vi "Build Toast With Classes.vi"(8 "error in":errorcluster) -> (0 "error out":errorcluster, 3 "Toast XML":string)   [LabVIEW 2026]
doc: "Interactive example using the public classes. Create a builder, add text, a Reply text input and a Reply button, inspect XML, initialize the service, register an injected ActivationHandler, then show the toast. Type a reply and click the toast button to inspect Arguments and User Inputs. Press Stop to unregister and close resources. A final System.GC.Collect call releases the callback reservation observed on this workstation; it is outside the callback. Running this VI displays a Windows notification and the example handler opens a blocking dialog."
uses:
  ActivationHandler/ActivationHandler.lvclass
  ToastBuilder/ToastBuilder.lvclass
  ToastService/ToastService.lvclass
panel:
  in  "stop":bool
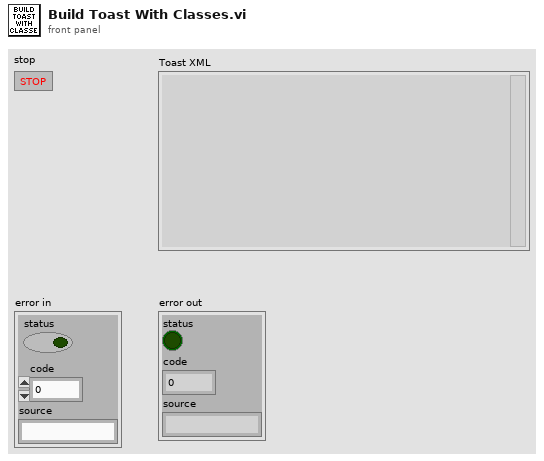
[diagram p1: front panel]
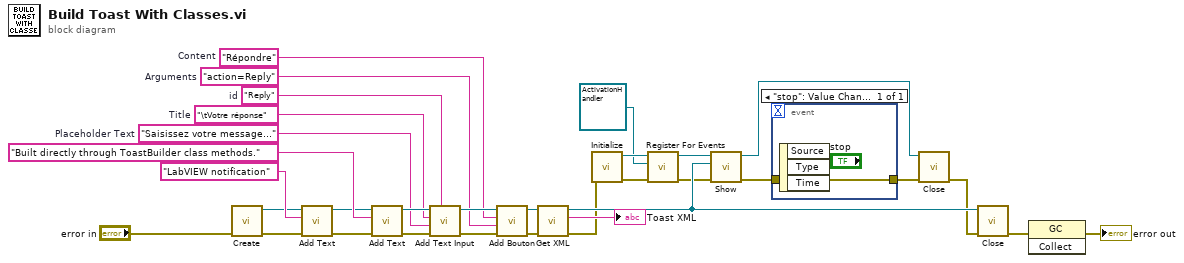
[diagram p0: block diagram]
diagram:
  w1 = "action=Reply"  # Arguments
  w2 = "Répondre"  # Content
  w7 = "Saisissez votre message…"  # Placeholder Text
  w8 = "\tVotre réponse"  # Title
  w9 = "Reply"  # id
  n1 = call "Create.vi"("error in"="error in") -> ("error out"=w27:errorcluster, "ToastBuilder out"=w26:refnum<class "ToastBuilder.lvclass">)  [unwired: 9 in]
  n2 = call "Add Text.vi"("error in"=w27, "text"="LabVIEW notification", "ToastBuilder in"=w26) -> ("error out"=w30:errorcluster, "ToastBuilder out"=w29:refnum<class "ToastBuilder.lvclass">)  [unwired: 7 in]
  n3 = call "Add Text.vi"("error in"=w30, "text"="Built directly through ToastBuilder class methods.", "ToastBuilder in"=w29) -> ("error out"=w10:errorcluster, "ToastBuilder out"=w11:refnum<class "ToastBuilder.lvclass">)  [unwired: 7 in]
  n4 = call "Add Text Input.vi"("id"=w9, "error in (no error)"=w10, "Placeholder Text"=w7, "Title"=w8, "ToastBuilder in"=w11) -> ("error out"=w6:errorcluster, "ToastBuilder out"=w4:refnum<class "ToastBuilder.lvclass">)  [unwired: 5 in]
  n5 = call "Add Bouton.vi"("error in (no error)"=w6, "Arguments"=w1, "Content"=w2, "ToastBuilder in"=w4) -> ("error out"=w5:errorcluster, "ToastBuilder out"=w3:refnum<class "ToastBuilder.lvclass">)  [unwired: 6 in]
  n6 = call "Get XML.vi"("error in"=w5, "ToastBuilder in"=w3) -> ("error out"=w23:errorcluster, "GetContent"=→"Toast XML":string, "ToastBuilder out"=w24:refnum<class "ToastBuilder.lvclass">)  [unwired: 7 in]
  n7 = call "Initialize.vi"("error in (no error)"=w23) -> ("error out"=w21:errorcluster, "ToastService out"=w19:refnum<class "ToastService.lvclass">)  [unwired: 9 in]
  n8 = call "Register For Events.vi"("error in (no error)"=w21, "ActivationHandler"=refnum<class "ActivationHandler.lvclass"> refnum, "ToastService in"=w19) -> ("error out"=w20:errorcluster, "ToastService out"=w18:refnum<class "ToastService.lvclass">)  [unwired: 7 in]
  n9 = call "Show.vi"("error in (no error)"=w20, "ToastBuilder in"=w24, "ToastService in"=w18) -> ("error out"=w16:errorcluster, "ToastService out"=w14:refnum<class "ToastService.lvclass">)  [unwired: 7 in]
  n10 = event shown="[0] \"stop\": Value Change" {
    selector: _ -> [_]
    dyn-events: _ -> [_]
    timeout: _ -> [_]
    tunnel: [w33] -> w15
    tunnel: w16 -> [w33]
    event "stop": Value Change {
      n11 = event-data() -> ()  [unwired: 1 in, 3 out]
    }
  }
  n12 = call "Close.vi"("error in (no error)"=w15, "ToastService in"=w14) -> ("error out"=w22:errorcluster)  [unwired: 9 in]
  n13 = call "Close.vi"("error in"=w22, "ToastBuilder in"=w24) -> ("error out"=w13:errorcluster)  [unwired: 9 in]
  n14 = invoke class="GC" method="Collect"(error in=w13) -> (error out=→"error out":errorcluster)  [unwired: 2 in, 2 out]
